vi "Evaluate Range Group.vi"(8 "error in":errorcluster, 10 "group":T1, 11 "num values":cluster{"channel":string, "value":dbl}[](array[cluster])) -> (0 "error out":errorcluster, 2 "first fail":string, 3 "passes":bool)   [LabVIEW 2026]
doc: "Range group over numeric IO values. Every 'and' item must be found and within [min,max]; at least one 'or' item must be found and within range (an empty 'or' list passes). An empty 'and' list passes. An unknown name fails and is reported."
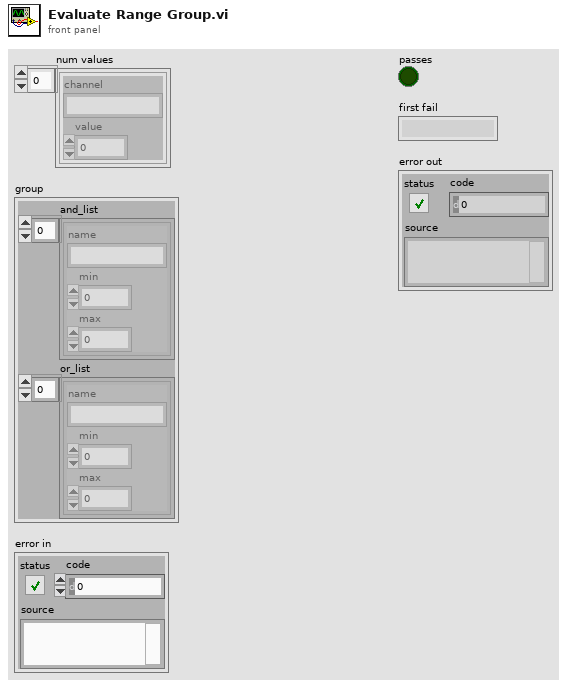
[diagram p1: front panel]
types:
  T1 = cluster{"and_list":cluster{"name":string, "min":dbl, "max":dbl}[], "or_list":cluster{"name":string, "min":dbl, "max":dbl}[]}
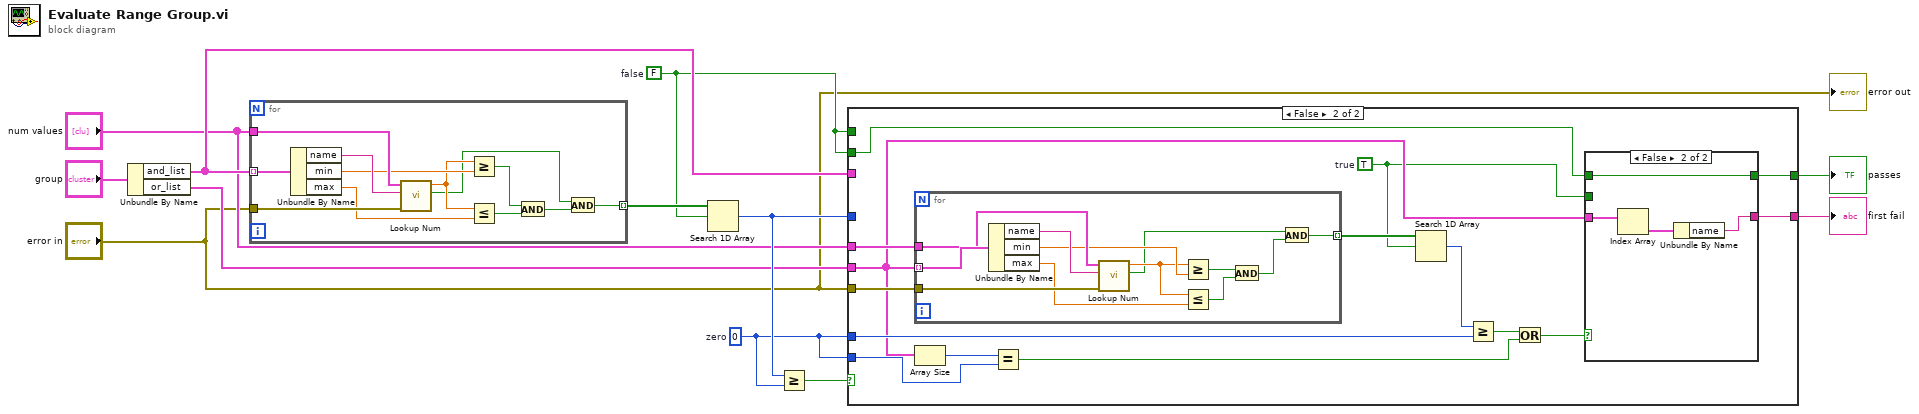
[diagram p0: block diagram]
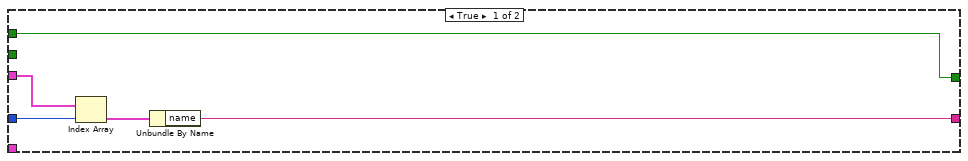
[diagram p2: hidden frame]
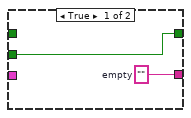
[diagram p3: hidden frame]
diagram:
  w6 = 0  # zero
  w5 = FALSE  # false
  n1 = Unbundle By Name("group") -> ("and_list"=w10:cluster{"name":string, "min":dbl, "max":dbl}[], "or_list"=w8:cluster{"name":string, "min":dbl, "max":dbl}[])
  n2 = for {
    tunnel: w10 -> [w24] mode=indexing
    tunnel: "num values" -> [w23]
    tunnel: "error in" -> [w21]
    tunnel: [w13] -> w11 mode=indexing
    n3 = Unbundle By Name(w24) -> ("name"=w22:string, "min"=w20:dbl, "max"=w18:dbl)
    n4 = call "Lookup Num.vi"("error in"=w21, "name"=w22, "num values"=w23) -> ("found"=w15:bool, "value"=w19:dbl)  [unwired: 6 in, 1 out]
    n5 = Greater Or Equal?(x=w19, y=w20) -> (x >= y?=w17:bool)
    n6 = Less Or Equal?(x=w19, y=w18) -> (x <= y?=w16:bool)
    n7 = And(x=w17, y=w16) -> (x .and. y?=w14:bool)
    n8 = And(x=w15, y=w14) -> (x .and. y?=w13:bool)
  }
  n9 = Search 1D Array(1D array=w11, element=w5) -> (index of element=w9:i32)  [unwired: 1 in]
  n10 = Greater Or Equal?(x=w9, y=w6) -> (x >= y?=w4:bool)
  n11 = case shown="False" w4 {
    tunnel: w10 -> [w29 _]
    tunnel: w9 -> [w28 _]
    tunnel: w8 -> [_ w35]
    tunnel: w5 -> [w26 _]
    tunnel: "num values" -> [_ w44]
    tunnel: "error in" -> [_ w43]
    tunnel: w6 -> [_ w38]
    tunnel: w6 -> [_ w41]
    tunnel: w5 -> [_ w33]
    tunnel: [w26 w31] -> w3
    tunnel: [w25 w30] -> w2
    frame True {
      n12 = Index Array(array=w29, index=w28) -> (element=w27:cluster{"name":string, "min":dbl, "max":dbl})
      n13 = Unbundle By Name(w27) -> ("name"=w25:string)
    }
    frame False {
      w34 = TRUE  # true
      n14 = for {
        tunnel: w35 -> [w62] mode=indexing
        tunnel: w44 -> [w61]
        tunnel: w43 -> [w59]
        tunnel: [w51] -> w40 mode=indexing
        n15 = Unbundle By Name(w62) -> ("name"=w60:string, "min"=w58:dbl, "max"=w56:dbl)
        n16 = call "Lookup Num.vi"("error in"=w59, "name"=w60, "num values"=w61) -> ("found"=w53:bool, "value"=w57:dbl)  [unwired: 6 in, 1 out]
        n17 = Greater Or Equal?(x=w57, y=w58) -> (x >= y?=w55:bool)
        n18 = Less Or Equal?(x=w57, y=w56) -> (x <= y?=w54:bool)
        n19 = And(x=w55, y=w54) -> (x .and. y?=w52:bool)
        n20 = And(x=w53, y=w52) -> (x .and. y?=w51:bool)
      }
      n21 = Array Size(array=w35) -> (size(s)=w42:i32)
      n22 = Equal?(x=w42, y=w41) -> (x = y?=w36:bool)
      n23 = Search 1D Array(1D array=w40, element=w34) -> (index of element=w39:i32)  [unwired: 1 in]
      n24 = Greater Or Equal?(x=w39, y=w38) -> (x >= y?=w37:bool)
      n25 = Or(x=w37, y=w36) -> (x .or. y?=w32:bool)
      n26 = case shown="False" w32 {
        tunnel: w35 -> [_ w50]
        tunnel: w34 -> [w46 _]
        tunnel: w33 -> [_ w48]
        tunnel: [w46 w48] -> w31
        tunnel: [w45 w47] -> w30
        frame True {
          w45 = ""  # empty
        }
        frame False {
          n27 = Index Array(array=w50) -> (element=w49:cluster{"name":string, "min":dbl, "max":dbl})  [unwired: 1 in]
          n28 = Unbundle By Name(w49) -> ("name"=w47:string)
        }
      }
    }
  }
  "passes" <- w3
  "first fail" <- w2
  "error out" <- "error in"
